vi "R r1p0s1b1.vi"(0 "x":dbl) -> (4 "y":dbl)   [LabVIEW 2026]
doc: "Reentrancy probe."
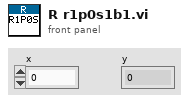
[diagram p1: front panel]
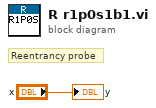
[diagram p0: block diagram]
diagram:
  # "Reentrancy probe"
  "y" <- "x"
